vi "timing accuracy.vi"() -> ()   [LabVIEW 2027]
uses:
  <vilib>/Analysis/NI_AALBase.lvlib
panel:
  out "variance":dbl
  out "std dev":dbl
  out "mean value":dbl
  out "Array":dbl[](array[numeric])
  out "Histogram Graph":T1(graph)
  in  "stop":bool
  in  "seconds to wait":dbl format="%#_6p"
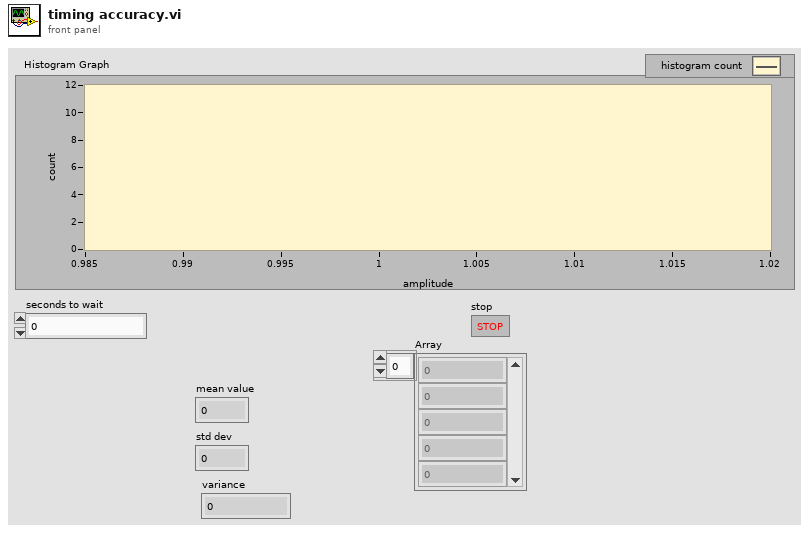
[diagram p1: front panel]
types:
  T1 = cluster{"X Values":dbl[], "Histogram: h(x)":i32[]}
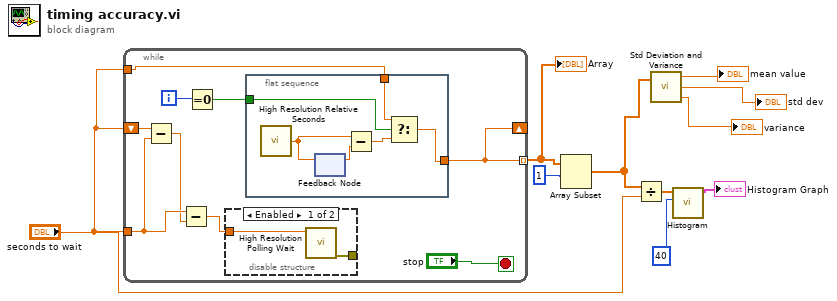
[diagram p0: block diagram]
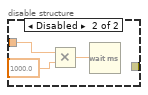
[diagram p2: hidden frame]
diagram:
  n1 = while {
    tunnel: [w18] -> w6 mode=indexing
    tunnel: "seconds to wait" -> [w16]
    shift-right: [w18] -> _
    shift-left: "seconds to wait" -> [w17]
    tunnel: "seconds to wait" -> [w11]
    i -> [w13]
    stop <- "stop" stop-if-true
    n2 = Subtract(x=w17, y=w16) -> (x-y=w15:dbl)
    n3 = Subtract(x=w16, y=w15) -> (x-y=w14:dbl)
    n4 = Equal To 0?(x=w13) -> (x = 0?=w12:bool)
    n5 = disable-structure shown="Enabled" {
      disable-tunnel: w14 -> [w21 w24]
      disable-tunnel: [w20 _] -> _
      frame Enabled {
        n6 = call <vilib>:"High Resolution Polling Wait.vi"("seconds to wait"=w21) -> ("error out"=w20:errorcluster)  [unwired: 10 in]
      }
      frame Disabled {
        n7 = Multiply(x=w24, y=1000.0) -> (x*y=w22:dbl)
        n8 = Wait (ms)(milliseconds to wait=w22) -> ()  [unwired: 1 out]
      }
    }
    n9 = flat-sequence {
      tunnel: [w26] -> w18
      tunnel: w12 -> [w28]
      tunnel: w11 -> [w25]
      frame #0 {
        n10 = call <vilib>:"High Resolution Relative Seconds.vi"() -> ("relative seconds"=w29:dbl)
        n11 = feedback #1() -> (w30:dbl)  [unwired: 1 in]
        n12 = feedback-in #1(w29) -> ()
        n13 = Subtract(x=w29, y=w30) -> (x-y=w27:dbl)
        n14 = Select(t=w25, s=w28, f=w27) -> (s? t:f=w26:dbl)
      }
    }
  }
  "Array" <- w6
  n15 = Array Subset(array=w6, index=1) -> (w4:dbl[])  [unwired: 1 in]
  n16 = Divide(x=w4, y="seconds to wait") -> (x/y=w8:dbl[])
  n17 = call <vilib>:"Std Deviation and Variance.vi"("X"=w4) -> ("mean"=→"mean value":dbl, "standard deviation"=→"std dev":dbl, "variance"=→"variance":dbl)  [unwired: 1 in]
  n18 = call <vilib>:"Histogram.vi"("intervals"=40, "X"=w8) -> ("Histogram Graph"=→"Histogram Graph":T1)  [unwired: 6 in, 3 out]
